vi "test2-ErrorStr conversion.vi"(8 "error in (no error)":errorcluster, 11 "TestCase in":refnum<class "testcase-CSMArgument.lvclass">) -> (0 "error out":errorcluster, 3 "TestCase out":refnum<class "testcase-CSMArgument.lvclass">)   [LabVIEW 2017, in "testcase-CSMArgument.lvclass"]
uses:
  testcase-CSMArgument.lvclass
  src/user.lib/_NEVSTOP/Communicable State Machine(CSM)/AdvanceAPI/CSM - Make String Arguments Safe.vi
  src/user.lib/_NEVSTOP/Communicable State Machine(CSM)/AdvanceAPI/CSM - Revert Arguments-Safe String.vi
  src/user.lib/_NEVSTOP/Communicable State Machine(CSM)/_Shared/Trim Single-line Text.vi
  src/user.lib/_NEVSTOP/Communicable State Machine(CSM)/AdvanceAPI/CSM - Keywords.vi
  <vilib>/addons/_JKI Toolkits/VI Tester/TestCase.llb/TestCase.lvclass
  src/user.lib/_NEVSTOP/Communicable State Machine(CSM)/Communicable State Machine.lvlib
  src/user.lib/_NEVSTOP/Communicable State Machine(CSM)/_Shared/CSM Shared.lvlib
  C:/Program Files (x86)/National Instruments/LabVIEW 2017/vi.lib/addons/_JKI Toolkits/VI Tester/TestCase.llb/TestCase.lvclass
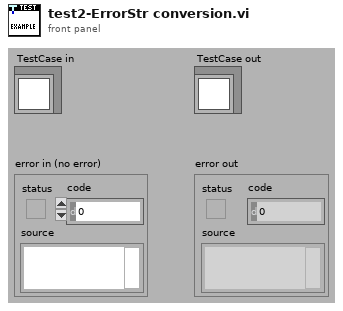
[diagram p1: front panel]
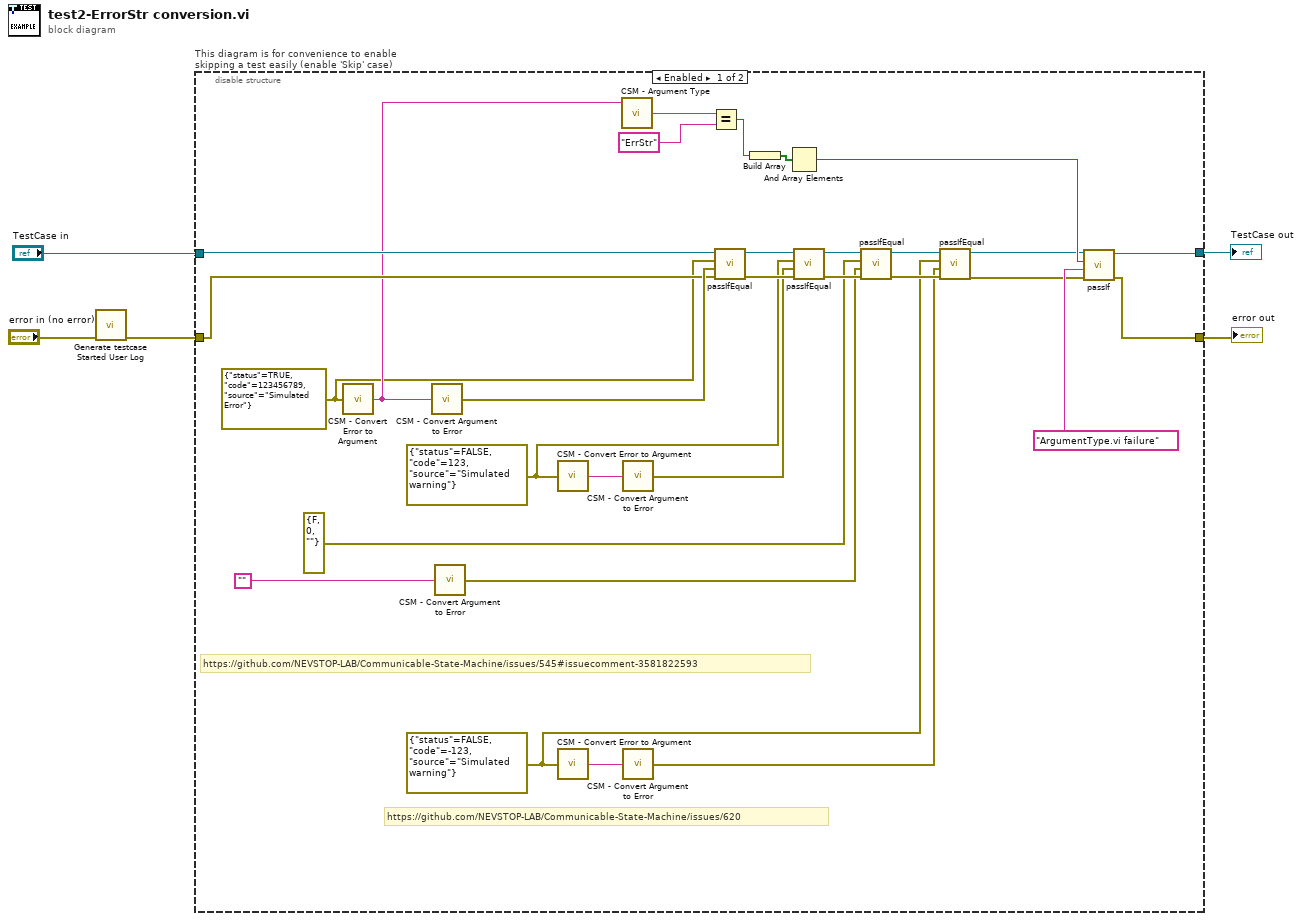
[diagram p0: block diagram]
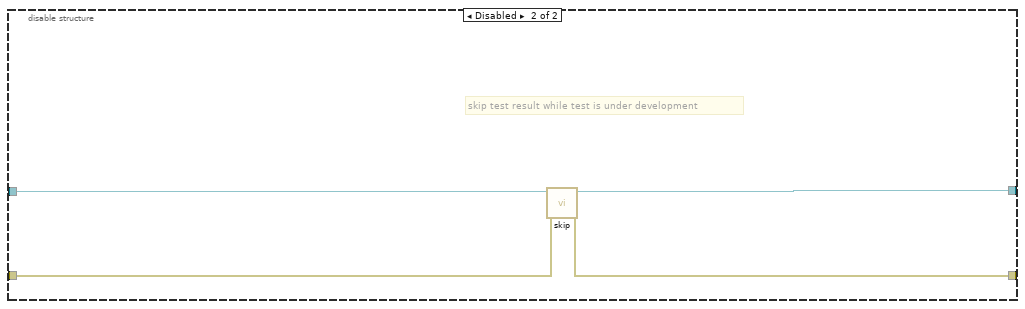
[diagram p2: hidden frame]
diagram:
  n1 = call "Generate testcase Started User Log.vi"("Error In"="error in (no error)") -> ("error out"=w1:errorcluster)  [unwired: 10 in]
  n2 = disable-structure "This diagram is for convenience to enable skipping a test easily (enable 'Skip' case)" shown="Enabled" {
    disable-tunnel: "TestCase in" -> [w35 w39]
    disable-tunnel: [w19 w37] -> w2
    disable-tunnel: [w20 w38] -> w4
    disable-tunnel: w1 -> [w29 w36]
    frame Enabled {
      w6 = errorcluster {"status"=FALSE, "code"=-123, "source"="Simulated warning"} ("error constant")
      w15 = errorcluster {"status"=FALSE, "code"=123, "source"="Simulated warning"} ("error constant")
      w13 = errorcluster {"status"=TRUE, "code"=123456789, "source"="Simulated Error"} ("error constant")
      # "https://github.com/NEVSTOP-LAB/Communicable-State-Machine/issues/620"
      # "https://github.com/NEVSTOP-LAB/Communicable-State-Machine/issues/545#issuecomment-3581822593"
      n3 = call "CSM - Convert Error to Argument.vi"("Error"=w13) -> ("Argument"=w22:string)  [unwired: 4 in]
      n4 = call "CSM - Convert Argument to Error.vi"("Argument"=w22) -> ("Error"=w30:errorcluster)  [unwired: 4 in]
      n5 = call "CSM - Convert Argument to Error.vi"("Argument"="") -> ("Error"=w26:errorcluster)  [unwired: 4 in]
      n6 = call "CSM - Convert Error to Argument.vi"("Error"=w15) -> ("Argument"=w21:string)  [unwired: 4 in]
      n7 = call "CSM - Convert Error to Argument.vi"("Error"=w6) -> ("Argument"=w12:string)  [unwired: 4 in]
      n8 = call "CSM - Argument Type.vi"("Arguments"=w22) -> ("Argument Type"=w23:string)  [unwired: 3 in, 1 out]
      n9 = call "CSM - Convert Argument to Error.vi"("Argument"=w21) -> ("Error"=w28:errorcluster)  [unwired: 4 in]
      n10 = call "CSM - Convert Argument to Error.vi"("Argument"=w12) -> ("Error"=w7:errorcluster)  [unwired: 4 in]
      n11 = Equal?(x=w23, y="ErrStr") -> (x = y?=w25:bool)
      n12 = call-dynamic "passIfEqual.vi"("error in (no error)"=w29, "y"=w30, "x"=w13, "TestCase in"=w35) -> ("error out"=w33:errorcluster, "TestCase out"=w34:refnum<class "testcase-CSMArgument.lvclass">)  [unwired: 6 in]
      n13 = Build Array(w25) -> (w24:bool[])
      n14 = And Array Elements(Boolean array=w24) -> (logical AND=w18:bool)
      n15 = call-dynamic "passIfEqual.vi"("error in (no error)"=w33, "y"=w28, "x"=w15, "TestCase in"=w34) -> ("error out"=w31:errorcluster, "TestCase out"=w32:refnum<class "testcase-CSMArgument.lvclass">)  [unwired: 6 in]
      n16 = call-dynamic "passIfEqual.vi"("error in (no error)"=w31, "y"=w26, "x"=errorcluster {"status"=FALSE, "code"=0, "source"=""} ("error constant"), "TestCase in"=w32) -> ("error out"=w11:errorcluster, "TestCase out"=w10:refnum<class "testcase-CSMArgument.lvclass">)  [unwired: 6 in]
      n17 = call-dynamic "passIfEqual.vi"("error in (no error)"=w11, "y"=w7, "x"=w6, "TestCase in"=w10) -> ("error out"=w8:errorcluster, "TestCase out"=w9:refnum<class "testcase-CSMArgument.lvclass">)  [unwired: 6 in]
      n18 = call-dynamic "passIf.vi"("error in (no error)"=w8, "message (\"\")"="ArgumentType.vi failure" ("message (\"\")"), "pass"=w18, "TestCase in"=w9) -> ("error out"=w20:errorcluster, "TestCase out"=w19:refnum<class "testcase-CSMArgument.lvclass">)  [unwired: 6 in]
    }
    frame Disabled {
      # "skip test result while test is under development"
      n19 = call <vilib>:"skip.vi"("error in (no error)"=w36, "TestCase in"=w39) -> ("error out"=w38:errorcluster, "TestCase out"=w37:refnum<class "testcase-CSMArgument.lvclass">)  [unwired: 8 in]
    }
  }
  "error out" <- w4
  "TestCase out" <- w2
